vi "test unknown method.vi"(8 "error in (no error)":errorcluster) -> (0 "error out":errorcluster, 3 "body":string)   [LabVIEW 2020, in "MCP Server tests.lvlib"]
doc: "A request with an unknown method must be answered with 200 and a JSON-RPC error with code -32601 (method not found) that carries the id of the request."
uses:
  MCP Server tests.lvlib
  <vilib>/JDP Science/JSONtext/Next JSON Value.vi
  <vilib>/JDP Science/JSONtext/String Subset.vi
  <vilib>/JDP Science/JSONtext/Parsing/Advance past next JSON Value (inlined COPY).vi
  <vilib>/JDP Science/JSONtext/Parsing/Advance past whitespace.vi
  <vilib>/JDP Science/JSONtext/Parsing/Advance past String.vi
  <vilib>/JDP Science/JSONtext/Parsing/Advance past Number.vi
  <vilib>/JDP Science/JSONtext/Parsing/Advance past Line Ending.vi
  <vilib>/JDP Science/JSONtext/Parsing/Parse Full Path or Item Name.vi
  <vilib>/JDP Science/JSONtext/Parsing/Advance past Array.vi
  <vilib>/JDP Science/JSONtext/Parsing/Advance past Object.vi
  <vilib>/JDP Science/JSONtext/support/Error Cluster From Code.vi
  <vilib>/JDP Science/JSONtext/Offset/Find Item Locations by Path.vi
  <vilib>/addons/_JKI Toolkits/Caraya/classes/Test/Test.lvclass
  <vilib>/JDP Science/JSONtext/JSONtext.lvlib
  <vilib>/addons/_JKI Toolkits/Caraya/classes/Assert/Assert.lvclass
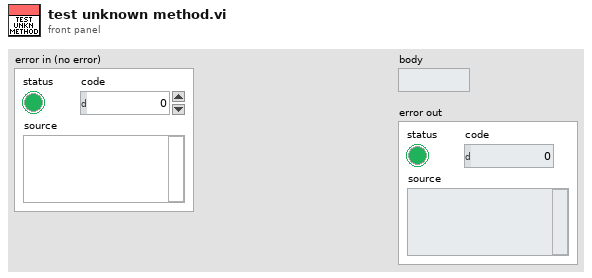
[diagram p1: front panel]
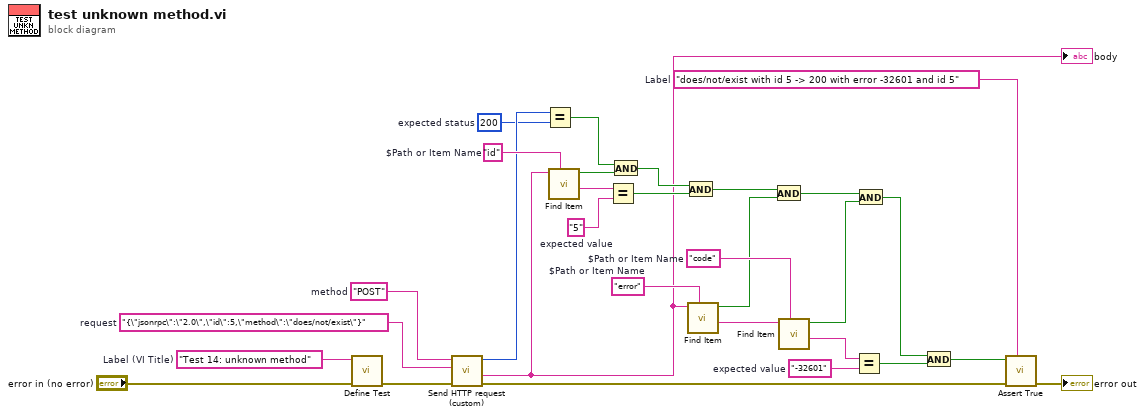
[diagram p0: block diagram]
diagram:
  w3 = "does/not/exist with id 5 -> 200 with error -32601 and id 5"  # Label
  w16 = "-32601"  # expected value
  w18 = "5"  # expected value
  w20 = 200  # expected status
  w22 = "code"  # $Path or Item Name
  w24 = "error"  # $Path or Item Name
  w25 = "id"  # $Path or Item Name
  w27 = "{\"jsonrpc\":\"2.0\",\"id\":5,\"method\":\"does/not/exist\"}"  # request
  w28 = "POST"  # method
  w30 = "Test 14: unknown method"  # Label (VI Title)
  n1 = call <vilib>:"Define Test.vi"("error in (no error)"="error in (no error)", "Label (VI Title)"=w30) -> ("error out"=w26:errorcluster)  [unwired: 8 in, 1 out]
  n2 = call "Send HTTP request (custom).vi"("error in (no error)"=w26, "request"=w27, "method"=w28) -> ("error out"=w4:errorcluster, "response"=w2:string, "status code"=w21:i32)  [unwired: 5 in, 1 out]
  "body" <- w2
  n3 = Equal?(x=w21, y=w20) -> (x = y?=w15:bool)
  n4 = call <vilib>:"Find Item.vi"("$Path or Item Name"=w25, "JSON"=w2) -> ("<JSON>"=w19:string, "Found"=w14:bool)  [unwired: 6 in, 2 out]
  n5 = Equal?(x=w19, y=w18) -> (x = y?=w12:bool)
  n6 = And(x=w15, y=w14) -> (x .and. y?=w13:bool)
  n7 = And(x=w13, y=w12) -> (x .and. y?=w11:bool)
  n8 = call <vilib>:"Find Item.vi"("$Path or Item Name"=w24, "JSON"=w2) -> ("<JSON>"=w23:string, "Found"=w10:bool)  [unwired: 6 in, 2 out]
  n9 = And(x=w11, y=w10) -> (x .and. y?=w9:bool)
  n10 = call <vilib>:"Find Item.vi"("$Path or Item Name"=w22, "JSON"=w23) -> ("<JSON>"=w17:string, "Found"=w8:bool)  [unwired: 6 in, 2 out]
  n11 = Equal?(x=w17, y=w16) -> (x = y?=w6:bool)
  n12 = And(x=w9, y=w8) -> (x .and. y?=w7:bool)
  n13 = And(x=w7, y=w6) -> (x .and. y?=w5:bool)
  n14 = call <vilib>:"Assert True.vi"("Label"=w3, "error in (no error)"=w4, "True?"=w5) -> ("error out"=→"error out":errorcluster)  [unwired: 7 in, 1 out]
